vi "Build HW Tree.vi"(8 "error in (no error)":errorcluster, 10 "HW Info":T1[](array[typedef]), 11 "Hardware Info Module in":refnum<class "Hardware Info Module.lvclass">) -> (0 "error out":errorcluster, 3 "Hardware Info Module out":refnum<class "Hardware Info Module.lvclass">)   [LabVIEW 2020, in "Volatus.lvlib" / "Hardware Info Module.lvclass"]
uses:
  Hardware Info Module.lvclass
  HW Info.ctl
  lv-cdm/CDM-Config/Config-JSON/Config-JSON.lvclass
  Hardware Info Module.lvclass/Hardware Info Module.ctl
  lv-cdm/CDM-Config/Config Manager/Config Manager.lvclass/Config Manager.ctl
  lv-cdm/CDM-Config/Config Element/Set Owner.vi
  lv-cdm/CDM-Config/Config Element/Config Element.lvclass
  lv-cdm/CDM-Config/Config Manager/Config Manager.lvclass
  <vilib>/JDP Science/JSONtext/JSONtext.lvlib
panel:
  out "JSON":string
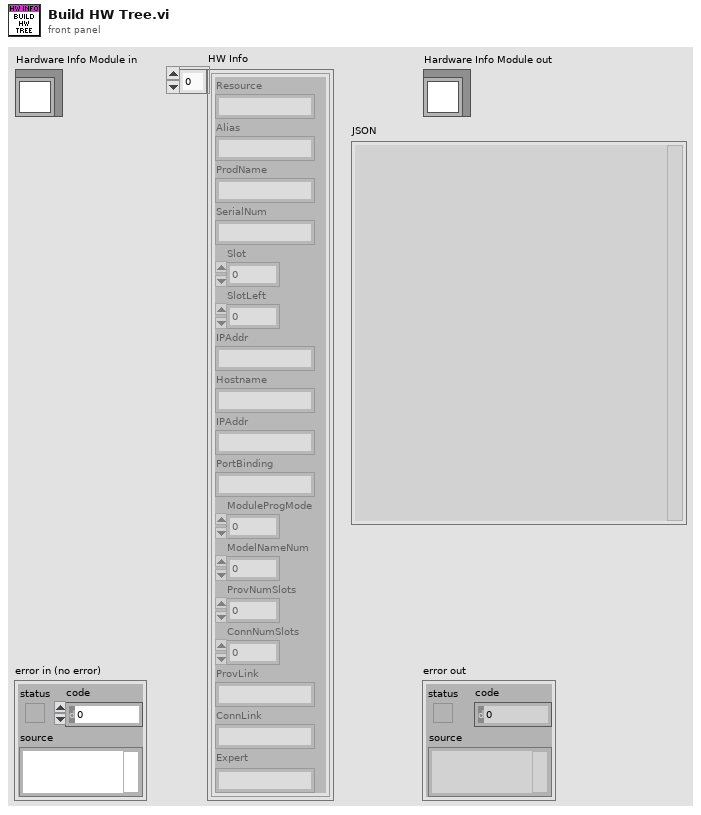
[diagram p1: front panel]
types:
  T1 = typedef "Volatus.lvlib/Hardware Info Module.lvclass/HW Info.ctl" = cluster{"Resource":string, "Alias":string, "ProdName":string, "SerialNum":string, "Slot":i32, "SlotLeft":u32, "IPAddr":string, "Hostname":string, "IPAddr":string, "PortBinding":string, "ModuleProgMode":u32, "ModelNameNum":u32, "ProvNumSlots":i32, "ConnNumSlots":i32, "ProvLink":string, "ConnLink":string, "Expert":string}
  T2 = typedef "Volatus.lvlib/Hardware Type.ctl" = enum16{"PC", "cRIO", "PXI"}
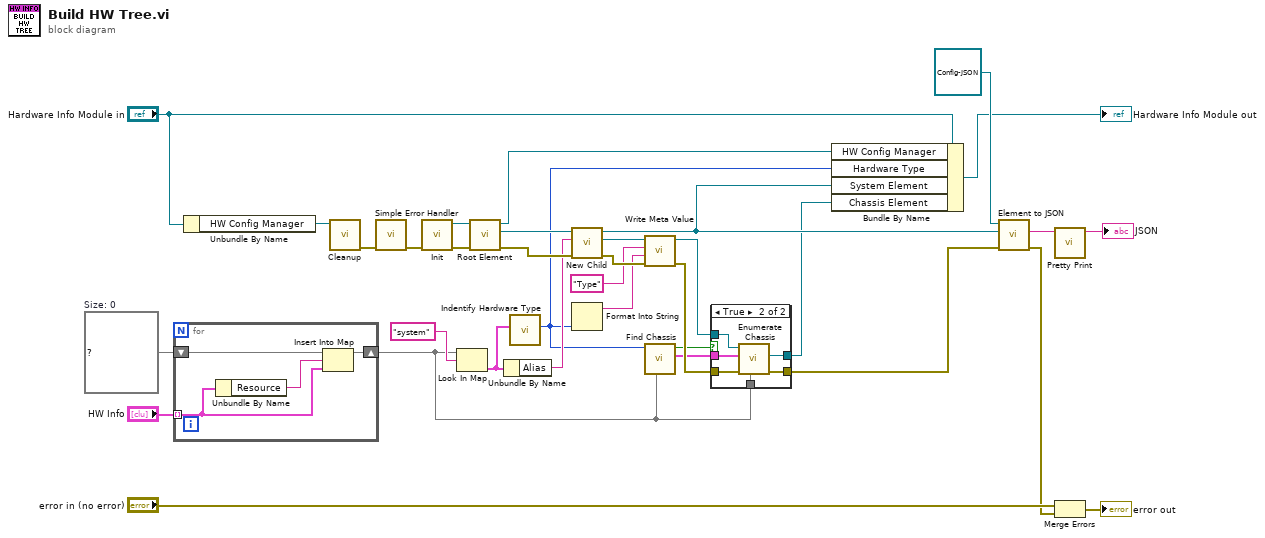
[diagram p0: block diagram]
diagram:
  w30 = map{string, T1} {}  # Size: 0
  n1 = for {
    shift-right: [w35] -> w7
    shift-left: w30 -> [w38]
    tunnel: "HW Info" -> [w36] mode=indexing
    n2 = Unbundle By Name(w36) -> ("Resource"=w37:string)
    n3 = Insert Into Map(map in=w38, key=w37, value=w36) -> (map out=w35:map{string, T1})  [unwired: 2 out]
  }
  n4 = Unbundle By Name("Hardware Info Module in") -> ("HW Config Manager"=w26:refnum<class "Config Manager.lvclass">)
  n5 = call "Cleanup.vi"("Config Manager in"=w26) -> ("error out"=w25:errorcluster)  [unwired: 10 in]
  n6 = call <vilib>:"Simple Error Handler.vi"("error in (no error)"=w25) -> ("error out"=w24:errorcluster)  [unwired: 4 in, 4 out]
  n7 = call "Init.vi"("error in (no error)"=w24) -> ("error out"=w16:errorcluster, "Config Manager out"=w23:refnum<class "Config Manager.lvclass">)  [unwired: 9 in]
  n8 = Look In Map(map=w7, key="system") -> (value=w20:T1)  [unwired: 1 in, 1 out]
  n9 = call "Root Element.vi"("error in (no error)"=w16, "Config Manager in"=w23) -> ("error out"=w33:errorcluster, "Root Element"=w22:refnum<class "Config Element.lvclass">, "Config Manager out"=w4:refnum<class "Config Manager.lvclass">)  [unwired: 7 in]
  n10 = Unbundle By Name(w20) -> ("Alias"=w21:string)
  n11 = call "Indentify Hardware Type.vi"("Hw Info"=w20) -> ("Hardware Type"=w5:T2)  [unwired: 8 in, 2 out]
  n12 = call "New Child.vi"("error in (no error)"=w33, "Child Name"=w21, "Config Element in"=w22) -> ("error out"=w32:errorcluster, "New Child"=w19:refnum<class "Config Element.lvclass">, "Config Element out"=w9:refnum<class "Config Element.lvclass">)  [unwired: 6 in]
  n13 = Format Into String(w5) -> (resulting string=w18:string)  [unwired: 3 in, 1 out]
  n14 = call "Write Meta Value.vi"("error in (no error)"=w32, "Meta Value"=w18, "Meta Name"="Type", "Config Element in"=w19) -> ("error out"=w34:errorcluster, "Config Element out"=w1:refnum<class "Config Element.lvclass">)  [unwired: 6 in]
  n15 = call "Find Chassis.vi"("Map"=w7, "Hardware Type"=w5) -> ("Chassis Info"=w8:T1, "Has Chassis"=w6:bool)  [unwired: 8 in]
  n16 = case shown="True" w6 {
    tunnel: w34 -> [w39 w45]
    tunnel: w1 -> [_ w44]
    tunnel: w8 -> [_ w43]
    tunnel: w7 -> [_ w42]
    tunnel: [w39 w41] -> w2
    tunnel: [_ w40] -> w3
    frame False {
    }
    frame True {
      n17 = call "Enumerate Chassis.vi"("Map"=w42, "error in (no error)"=w45, "Chassis Info"=w43, "System Element"=w44) -> ("error out"=w41:errorcluster, "Chassis Element"=w40:refnum<class "Config Element.lvclass">)  [unwired: 6 in]
    }
  }
  n18 = Bundle By Name(cluster="Hardware Info Module in", "HW Config Manager"=w4, "Hardware Type"=w5, "System Element"=w9, "Chassis Element"=w3) -> (→"Hardware Info Module out":refnum<class "Hardware Info Module.lvclass">)
  n19 = call "Element to JSON.vi"("error in (no error)"=w2, "Element"=w9, "Config-JSON"=refnum<class "Config-JSON.lvclass"> refnum) -> ("error out"=w12:errorcluster, "JSON"=w15:string)  [unwired: 7 in]
  n20 = call <vilib>:"Pretty Print.vi"("JSON"=w15) -> ("<JSON>"=→"JSON":string)  [unwired: 8 in, 2 out]
  n21 = Merge Errors("error in (no error)", w12) -> (→"error out":errorcluster)
